vi "A.vi"(0 "x":dbl, 11 "error in":errorcluster) -> (4 "y":dbl, 15 "error out":errorcluster)   [LabVIEW 2026]
doc: "Repro callee: adds one to x."
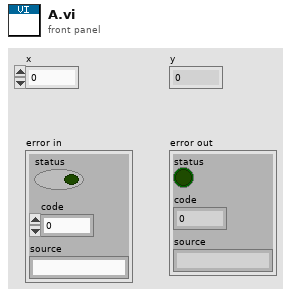
[diagram p1: front panel]
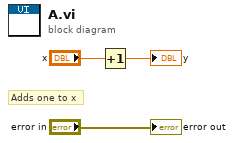
[diagram p0: block diagram]
diagram:
  # "Adds one to x"
  n1 = Increment(x="x") -> (x+1=→"y":dbl)
  "error out" <- "error in"
